vi "Measure4.vi"() -> ()   [LabVIEW 2024]
uses:
  <vilib>/MakerHub/LINX/Public/Peripherals/Analog/Analog Read N Chans.vi
  <vilib>/MakerHub/LINX/Public/Peripherals/PWM/PWM Set Duty Cycle 1 Chan.vi
  <vilib>/MakerHub/LINX/Public/Peripherals/Digital/Digital Read 1 Chan.vi
  <vilib>/MakerHub/LINX/Private/Local IO/LinxAnalogRead.vi
  <vilib>/MakerHub/LINX/Public/Utilities/Check Channel.vi
  <vilib>/MakerHub/LINX/Public/Peripherals/Digital/Digital Read N Chans.vi
  <vilib>/MakerHub/LINX/Private/Local IO/LinxDigitalRead.vi
  <vilib>/MakerHub/LINX/Public/Utilities/Open Serial.vi
  Globals.vi
  <vilib>/MakerHub/LINX/Public/Peripherals/PWM/PWM Set Duty Cycle N Chans.vi
  <vilib>/addons/control/pid/pid.llb/PID (DBL).vi
  <vilib>/MakerHub/LINX/Private/Utilties/Generate Error.vi
  <vilib>/Utility/file.llb/Write Delimited Spreadsheet (string).vi
  <vilib>/MakerHub/LINX/LMH-LINX.lvlib
  <vilib>/addons/control/pid/NI_PID_pid.lvlib
  <vilib>/Analysis/NI_AALBase.lvlib
panel:
  out "A5":dbl
  out "Resistance Amplified":dbl
  out "Resistance A3":dbl
  in  "Current":dbl
  out "A2 (TH)":dbl
  out "A1 (Voltage)":dbl
  out "A0 (TC)":dbl
  out "Resistance Amplified":dbl(graph)
  out "A4":dbl
  out "A3":dbl
  out "Resistance A3":dbl(graph)
  out "TREF 2 Error":dbl
  out "TREF 2":dbl
  out "TREF 1 Error":dbl
  out "Seebeck Coeff":dbl
  out "TREF 1":dbl
  in  "Target TC":dbl format="%.2f"
  in  "Target TH":dbl format="%.2f"
  out "Auto":bool
  in  "Start Auto":bool
  in  "TH End":dbl(knob)=100.0 step=10.0 scale=0.0..100.0
  in  "TH Start":dbl(knob)=40.0 step=10.0 scale=0.0..100.0
  out "VOUT - 1.25":dbl(knob) scale=-1.0..1.0
  out "TC":dbl(slide) scale=0.0..100.0
  out "TH":dbl(slide) scale=0.0..100.0
  out "Voltage":dbl(graph)
  out "TH":dbl(graph)
  in  "Save to File":bool
  out "VOUT - 1.25":dbl
  out "TC":dbl(graph)
  out "TC":dbl
  in  "Stop Button":bool
  out "TH":dbl
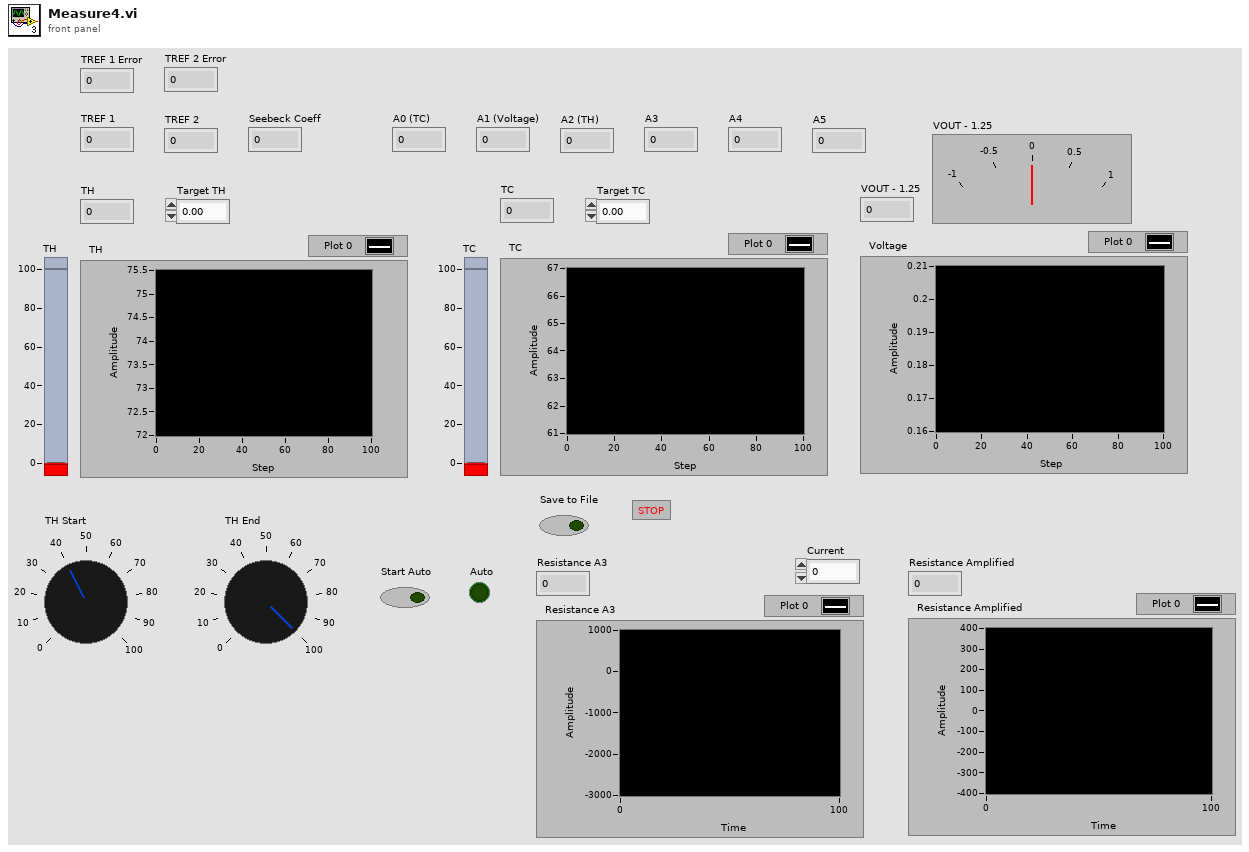
[diagram p1: front panel]
types:
  T1 = typedef "LMH-LINX.lvlib/LINX Ref.ctl" = cluster{"IO":T2, "Interface":T3, "LINX Device Config":T4}
  T2 = typedef "LMH-LINX.lvlib/Platform.ctl" = enum16{"Remote", "Local"}
  T3 = typedef "LMH-LINX.lvlib/Interface.ctl" = enum16{"Serial", "TCP"}
  T4 = typedef "LMH-LINX.lvlib/Device.lvlib/LINX Device Config.ctl" = cluster{"Interface":T3, "COM Port":refnum<visa-resource-name>, "TCP Configuration":T5, "Device Family":u8, "Device ID":u8, "Device Name":string, "TCP Ref":refnum<k5>, "Channels":T6}
  T5 = typedef "LMH-LINX.lvlib/Device.lvlib/TCP Config.ctl" = cluster{"IP Address":string, "Port":u16}
  T6 = typedef "LMH-LINX.lvlib/Channels.ctl" = cluster{"DI":u8[], "DO":u8[], "AI":u8[], "AO":u8[], "PWM":u8[], "QE":u8[], "UART":u8[], "I2C 2":u8[], "SPI":u8[], "CAN":u8[], "Servo":u8[], "AI Ref (V)":dbl, "AI Resolution (Bits)":u8, "AO Ref (V)":dbl, "AO Resolution (Bits)":u8}
  T7 = cluster{"proportional gain (Kc)":dbl, "integral time (Ti, min)":dbl, "derivative time (Td, min)":dbl}
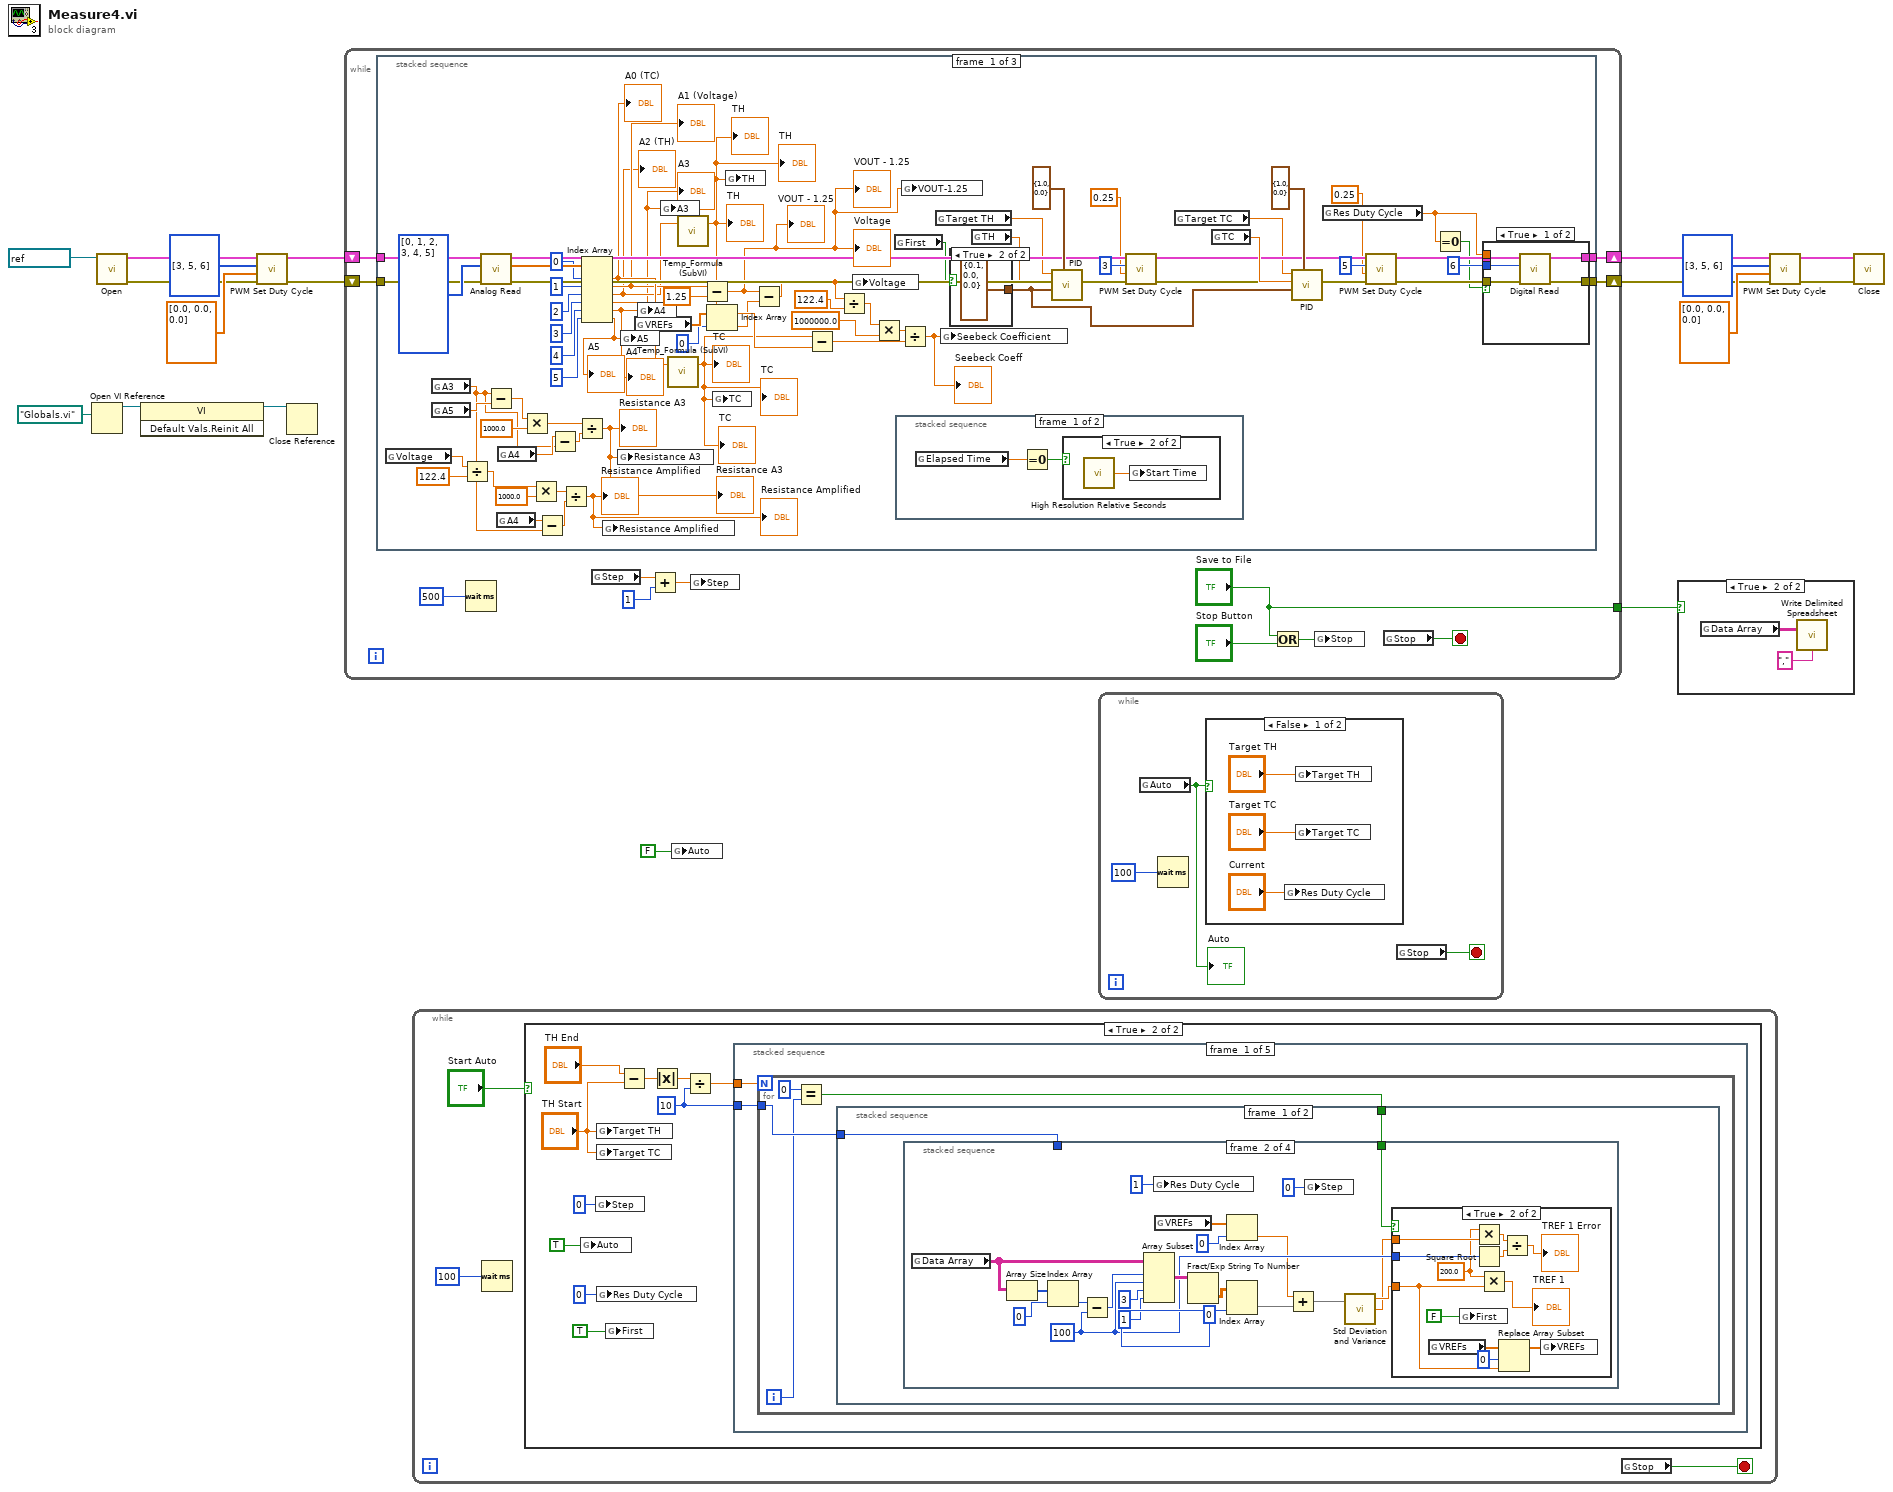
[diagram p0: block diagram]
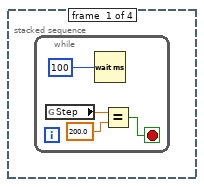
[diagram p3: hidden frame]
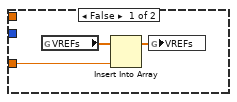
[diagram p4: hidden frame]
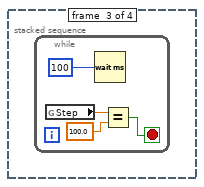
[diagram p5: hidden frame]
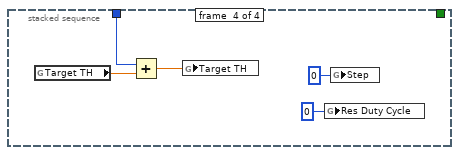
[diagram p6: hidden frame]
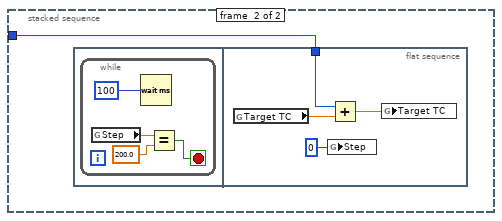
[diagram p7: hidden frame]
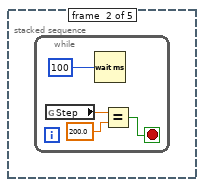
[diagram p8: hidden frame]
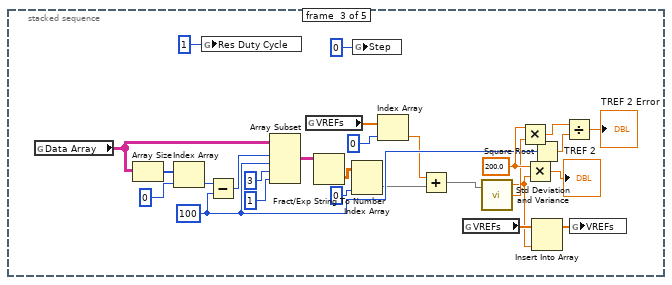
[diagram p9: hidden frame]
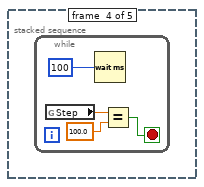
[diagram p10: hidden frame]
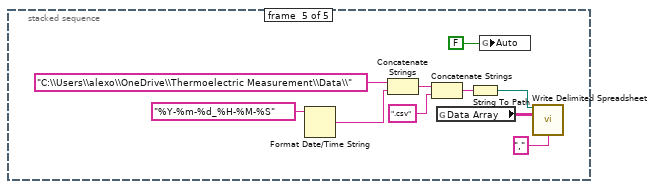
[diagram p11: hidden frame]
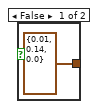
[diagram p14: hidden frame]
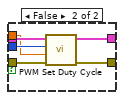
[diagram p15: hidden frame]
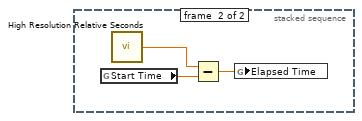
[diagram p17: hidden frame]
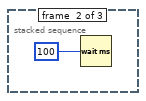
[diagram p18: hidden frame]
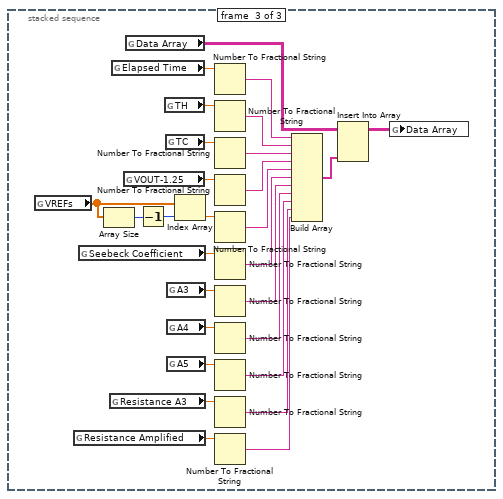
[diagram p19: hidden frame]
diagram:
  n1 = Open VI Reference(vi path=path "Globals.vi") -> (vi reference=w16:refnum<vi>)  [unwired: 5 in, 1 out]
  n2 = call-poly <vilib>:"Open.vi"("Serial Port"=refnum<visa-resource-name> "COM7") -> ("Error Out"=w8:errorcluster, "LINX Resource"=w11:T1)  [unwired: 8 in, 1 out]
  n3 = invoke class="VI" method="Default Vals.Reinit All"(reference=w16) -> (reference out=w15:refnum<vi>)  [unwired: 2 in, 2 out]
  n4 = call-poly <vilib>:"PWM Set Duty Cycle.vi"("Error In"=w8, "Duty Cycles"=dbl[] [0.0, 0.0, 0.0] ("Duty Cycle (0-1)"), "PWM Channels"=u8[] [3, 5, 6] ("PWM Channel"), "LINX Resource"=w11) -> ("Error Out"=w7:errorcluster, "LINX Resource"=w12:T1)  [unwired: 6 in]
  n5 = Close Reference(reference=w15) -> ()  [unwired: 1 in, 1 out]
  n6 = while {
    shift-right: [w29] -> w4
    shift-left: w12 -> [w30]
    shift-right: [w27] -> w1
    shift-left: w7 -> [w28]
    tunnel: ["Save to File"] -> w17
    stop <- w22 stop-if-true
    n7 = stacked-sequence {
      tunnel: w30 -> [w90 _ _]
      tunnel: [w56 _ _] -> w29
      tunnel: w28 -> [w89 _ _]
      tunnel: [w54 _ _] -> w27
      frame #0 {
        n8 = global read "Globals.vi" "Voltage"() -> (w52:dbl)
        n9 = global read "Globals.vi" "A3"() -> (w33:dbl)
        n10 = global read "Globals.vi" "A5"() -> (w41:dbl)
        n11 = Divide(x=w52, y=122.4) -> (x/y=w36:dbl)
        n12 = call-poly <vilib>:"Analog Read.vi"("Error In"=w89, "AI Channel(s)"=i32[] [0, 1, 2, 3, 4, 5], "LINX Resource"=w90) -> ("Error Out"=w87:errorcluster, "Voltages"=w96:dbl[], "LINX Resource"=w88:T1)  [unwired: 5 in, 1 out]
        n13 = Subtract(x=w33, y=w41) -> (x-y=w39:dbl)
        n14 = global read "Globals.vi" "A4"() -> (w37:dbl)
        n15 = global read "Globals.vi" "A4"() -> (w38:dbl)
        n16 = Multiply(x=w39, y=1000.0) -> (x*y=w67:dbl)
        n17 = Multiply(x=w36, y=1000.0) -> (x*y=w62:dbl)
        n18 = Subtract(x=w37, y=w33) -> (x-y=w61:dbl)
        n19 = Subtract(x=w38, y=w33) -> (x-y=w63:dbl)
        n20 = Divide(x=w62, y=w61) -> (x/y=w50:dbl)
        "Resistance Amplified" <- w50
        "Resistance Amplified" <- w50
        n21 = Divide(x=w67, y=w63) -> (x/y=w51:dbl)
        "Resistance A3" <- w51
        "Resistance A3" <- w51
        n22 = Index Array(array=w96, index #1=0 ("index"), index #2=1 ("index"), index #3=2 ("index"), index #4=3 ("index"), index #5=4 ("index"), index #6=5 ("index")) -> (element #1=w60:dbl, element #2=w59:dbl, element #3=w58:dbl, element #4=w48:dbl, element #5=w47:dbl, element #6=w43:dbl)
        "A3" <- w48
        "A4" <- w47
        "A0 (TC)" <- w60
        "A1 (Voltage)" <- w59
        "A2 (TH)" <- w58
        "A5" <- w43
        n23 = global write "Globals.vi" "Resistance Amplified"(w50) -> ()
        n24 = global write "Globals.vi" "Resistance A3"(w51) -> ()
        n25 = global write "Globals.vi" "A5"(w43) -> ()
        n26 = global read "Globals.vi" "VREFs"() -> (w71:dbl[])
        n27 = global write "Globals.vi" "A4"(w47) -> ()
        n28 = global write "Globals.vi" "A3"(w48) -> ()
        n29 = call "Temp_Formula (SubVI).vi"("In"=w60) -> ("Out"=w72:dbl)  [unwired: 1 in, 1 out]
        "TC" <- w72
        "TC" <- w72
        "TC" <- w72
        n30 = call "Temp_Formula (SubVI).vi"("In"=w58) -> ("Out"=w73:dbl)  [unwired: 1 in, 1 out]
        "TH" <- w73
        "TH" <- w73
        "TH" <- w73
        n31 = Subtract(x=w59, y=1.25) -> (x-y=w49:dbl)
        "VOUT - 1.25" <- w49
        "Voltage" <- w49
        "VOUT - 1.25" <- w49
        n32 = Index Array(array=w71, index=0) -> (element=w69:dbl)
        n33 = global write "Globals.vi" "TC"(w72) -> ()
        n34 = global write "Globals.vi" "TH"(w73) -> ()
        n35 = Subtract(x=w49, y=w69) -> (x-y=w68:dbl)
        n36 = Subtract(x=w72, y=w73) -> (x-y=w99:dbl)
        n37 = Divide(x=w68, y=122.4) -> (x/y=w74:dbl)
        n38 = global write "Globals.vi" "Voltage"(w68) -> ()
        n39 = Multiply(x=w74, y=1000000.0) -> (x*y=w77:dbl)
        n40 = global read "Globals.vi" "First"() -> (w35:bool)
        n41 = stacked-sequence {
          frame #0 {
            n42 = global read "Globals.vi" "Elapsed Time"() -> (w113:dbl)
            n43 = Equal To 0?(x=w113) -> (x = 0?=w114:bool)
            n44 = case shown="True" w114 {
              frame False {
              }
              frame True {
                n45 = call <vilib>:"High Resolution Relative Seconds.vi"() -> ("relative seconds"=w115:dbl)
                n46 = global write "Globals.vi" "Start Time"(w115) -> ()
              }
            }
          }
          frame #1 {
            n47 = global read "Globals.vi" "Start Time"() -> (w116:dbl)
            n48 = call <vilib>:"High Resolution Relative Seconds.vi"() -> ("relative seconds"=w117:dbl)
            n49 = Subtract(x=w117, y=w116) -> (x-y=w118:dbl)
            n50 = global write "Globals.vi" "Elapsed Time"(w118) -> ()
          }
        }
        n51 = Divide(x=w77, y=w99) -> (x/y=w98:dbl)
        "Seebeck Coeff" <- w98
        n52 = global write "Globals.vi" "VOUT-1.25"(w49) -> ()
        n53 = global read "Globals.vi" "Target TH"() -> (w80:dbl)
        n54 = global write "Globals.vi" "Seebeck Coefficient"(w98) -> ()
        n55 = case shown="True" w35 {
          tunnel: [T7 {"proportional gain (Kc)"=0.01, "integral time (Ti, min)"=0.14, "derivative time (Td, min)"=0.0} ("PID gains") T7 {"proportional gain (Kc)"=0.1, "integral time (Ti, min)"=0.0, "derivative time (Td, min)"=0.0} ("PID gains")] -> w34
          frame False {
          }
          frame True {
          }
        }
        n56 = global read "Globals.vi" "TH"() -> (w86:dbl)
        n57 = call-poly <vilib>:"PID.vi"("output range"=cluster{"output high":dbl, "output low":dbl} {"output high"=1.0, "output low"=0.0}, "PID gains"=w34, "process variable"=w86, "setpoint"=w80) -> ()  [unwired: 6 in, 2 out]
        n58 = call-poly <vilib>:"PWM Set Duty Cycle.vi"("Error In"=w87, "Duty Cycle (0-1)"=0.25, "PWM Channel"=u8 3, "LINX Resource"=w88) -> ("Error Out"=w81:errorcluster, "LINX Resource"=w82:T1)  [unwired: 6 in]
        n59 = global read "Globals.vi" "Target TC"() -> (w79:dbl)
        n60 = global read "Globals.vi" "TC"() -> (w83:dbl)
        n61 = call-poly <vilib>:"PID.vi"("output range"=cluster{"output high":dbl, "output low":dbl} {"output high"=1.0, "output low"=0.0}, "PID gains"=w34, "process variable"=w83, "setpoint"=w79) -> ()  [unwired: 6 in, 2 out]
        n62 = global read "Globals.vi" "Res Duty Cycle"() -> (w46:dbl)
        n63 = call-poly <vilib>:"PWM Set Duty Cycle.vi"("Error In"=w81, "Duty Cycle (0-1)"=0.25, "PWM Channel"=u8 5, "LINX Resource"=w82) -> ("Error Out"=w55:errorcluster, "LINX Resource"=w57:T1)  [unwired: 6 in]
        n64 = Equal To 0?(x=w46) -> (x = 0?=w45:bool)
        n65 = case shown="True" w45 {
          tunnel: w57 -> [w106 w112]
          tunnel: [w105 w111] -> w56
          tunnel: w55 -> [w103 w110]
          tunnel: [w104 w109] -> w54
          tunnel: u8 6 ("PWM Channel") -> [w102 w108]
          tunnel: w46 -> [_ w107]
          frame True {
            n66 = call-poly <vilib>:"Digital Read.vi"("Error In"=w103, "DI Channel"=w102, "LINX Resource"=w106) -> ("Error Out"=w104:errorcluster, "LINX Resource"=w105:T1)  [unwired: 6 in, 1 out]
          }
          frame False {
            n67 = call-poly <vilib>:"PWM Set Duty Cycle.vi"("Error In"=w110, "Duty Cycle (0-1)"=w107, "PWM Channel"=w108, "LINX Resource"=w112) -> ("Error Out"=w109:errorcluster, "LINX Resource"=w111:T1)  [unwired: 6 in]
          }
        }
      }
      frame #1 {
        n68 = Wait (ms)(milliseconds to wait=u32 100) -> ()  [unwired: 1 out]
      }
      frame #2 {
        n69 = global read "Globals.vi" "VREFs"() -> (w134:dbl[])
        n70 = global read "Globals.vi" "Resistance Amplified"() -> (w121:dbl)
        n71 = global read "Globals.vi" "Seebeck Coefficient"() -> (w138:dbl)
        n72 = Array Size(array=w134) -> (size(s)=w133:i32)
        n73 = global read "Globals.vi" "Resistance A3"() -> (w125:dbl)
        n74 = global read "Globals.vi" "Elapsed Time"() -> (w136:dbl)
        n75 = global read "Globals.vi" "VOUT-1.25"() -> (w143:dbl)
        n76 = global read "Globals.vi" "Data Array"() -> (w146:string[][])
        n77 = Decrement(x=w133) -> (x-1=w132:i32)
        n78 = global read "Globals.vi" "TH"() -> (w139:dbl)
        n79 = global read "Globals.vi" "TC"() -> (w141:dbl)
        n80 = global read "Globals.vi" "A3"() -> (w126:dbl)
        n81 = global read "Globals.vi" "A4"() -> (w127:dbl)
        n82 = global read "Globals.vi" "A5"() -> (w124:dbl)
        n83 = Index Array(array=w134, index=w132) -> (element=w131:dbl)
        n84 = Number To Fractional String(number=w136) -> (F-format string=w137:string)  [unwired: 3 in]
        n85 = Number To Fractional String(number=w139) -> (F-format string=w140:string)  [unwired: 3 in]
        n86 = Number To Fractional String(number=w141) -> (F-format string=w142:string)  [unwired: 3 in]
        n87 = Number To Fractional String(number=w143) -> (F-format string=w144:string)  [unwired: 3 in]
        n88 = Number To Fractional String(number=w131) -> (F-format string=w130:string)  [unwired: 3 in]
        n89 = Number To Fractional String(number=w138) -> (F-format string=w135:string)  [unwired: 3 in]
        n90 = Number To Fractional String(number=w126) -> (F-format string=w129:string)  [unwired: 3 in]
        n91 = Number To Fractional String(number=w127) -> (F-format string=w128:string)  [unwired: 3 in]
        n92 = Number To Fractional String(number=w124) -> (F-format string=w123:string)  [unwired: 3 in]
        n93 = Number To Fractional String(number=w125) -> (F-format string=w122:string)  [unwired: 3 in]
        n94 = Number To Fractional String(number=w121) -> (F-format string=w120:string)  [unwired: 3 in]
        n95 = Build Array(w137, w140, w142, w144, w130, w135, w129, w128, w123, w122, w120) -> (w145:string[])
        n96 = Insert Into Array(array=w146, new element=w145) -> (w147:string[][])  [unwired: 2 in]
        n97 = global write "Globals.vi" "Data Array"(w147) -> ()
      }
    }
    n98 = Wait (ms)(milliseconds to wait=u32 500) -> ()  [unwired: 1 out]
    n99 = global read "Globals.vi" "Step"() -> (w21:dbl)
    n100 = Add(x=w21, y=1) -> (x+y=w20:dbl)
    n101 = global write "Globals.vi" "Step"(w20) -> ()
    n102 = Or(x="Save to File", y="Stop Button") -> (x .or. y?=w23:bool)
    n103 = global write "Globals.vi" "Stop"(w23) -> ()
    n104 = global read "Globals.vi" "Stop"() -> (w22:bool)
  }
  n105 = while {
    stop <- w149 stop-if-true
    n106 = Wait (ms)(milliseconds to wait=u32 100) -> ()  [unwired: 1 out]
    n107 = case shown="True" "Start Auto" {
      frame False {
      }
      frame True {
        w155 = 10
        n108 = global write "Globals.vi" "Auto"(TRUE) -> ()
        n109 = global write "Globals.vi" "Step"(0) -> ()
        n110 = global write "Globals.vi" "Target TH"("TH Start") -> ()
        n111 = global write "Globals.vi" "Target TC"("TH Start") -> ()
        n112 = global write "Globals.vi" "Res Duty Cycle"(0) -> ()
        n113 = global write "Globals.vi" "First"(TRUE) -> ()
        n114 = Subtract(x="TH End", y="TH Start") -> (x-y=w158:dbl)
        n115 = Absolute Value(x=w158) -> (abs(x)=w157:dbl)
        n116 = Divide(x=w157, y=w155) -> (x/y=w154:dbl)
        n117 = stacked-sequence {
          tunnel: w154 -> [w162 _ _ _ _]
          tunnel: w155 -> [w161 _ _ _ _]
          frame #0 {
            n118 = for {
              N: w162 -> [_]
              tunnel: w161 -> [w166]
              i -> [w163]
              n119 = Equal?(x=0 ("y"), y=w163) -> (x = y?=w165:bool)
              n120 = stacked-sequence {
                tunnel: w166 -> [w168 w218]
                tunnel: w165 -> [w167 _]
                frame #0 {
                  n121 = stacked-sequence {
                    tunnel: w168 -> [_ _ _ w215]
                    tunnel: w167 -> [_ w193 _ _]
                    frame #0 {
                      n122 = while {
                        stop <- w169 stop-if-true
                        n123 = global read "Globals.vi" "Step"() -> (w171:dbl)
                        n124 = Wait (ms)(milliseconds to wait=u32 100) -> ()  [unwired: 1 out]
                        n125 = Equal?(x=w171, y=200.0) -> (x = y?=w169:bool)
                      }
                    }
                    frame #1 {
                      w181 = 100 ("y")
                      n126 = global read "Globals.vi" "Data Array"() -> (w187:string[][])
                      n127 = Array Size(array=w187) -> (size(s)=w188:i32[])
                      n128 = Index Array(array=w188, index=0) -> (element=w189:i32)
                      n129 = Subtract(x=w189, y=w181) -> (x-y=w190:i32)
                      n130 = Array Subset(array=w187, index (row)=w190, length (row)=w181, index (col)=3 ("index"), length (col)=1 ("length")) -> (w191:string[][])
                      n131 = global write "Globals.vi" "Res Duty Cycle"(1) -> ()
                      n132 = global read "Globals.vi" "VREFs"() -> (w179:dbl[])
                      n133 = Fract/Exp String To Number(string=w191) -> (number=w192:dbl[][])  [unwired: 3 in, 1 out]
                      n134 = Index Array(array=w179, index=0) -> (element=w177:dbl)
                      n135 = Index Array(array=w192, index (col)=0 ("dimension size")) -> (element=w175:dbl[])  [unwired: 1 in]
                      n136 = Add(x=w177, y=w175) -> (x+y=w176:dbl[])
                      n137 = global write "Globals.vi" "Step"(0) -> ()
                      n138 = call <vilib>:"Std Deviation and Variance.vi"("X"=w176) -> ("mean"=w182:dbl, "standard deviation"=w180:dbl)  [unwired: 1 in, 1 out]
                      n139 = case shown="True" w193 {
                        tunnel: w182 -> [w194 w199]
                        tunnel: w181 -> [_ w206]
                        tunnel: w180 -> [_ w205]
                        frame False {
                          n140 = global read "Globals.vi" "VREFs"() -> (w195:dbl[])
                          n141 = Insert Into Array(array=w195, new element=w194) -> (w196:dbl[])  [unwired: 1 in]
                          n142 = global write "Globals.vi" "VREFs"(w196) -> ()
                        }
                        frame True {
                          w202 = 200.0 ("x")
                          n143 = global read "Globals.vi" "VREFs"() -> (w201:dbl[])
                          n144 = global write "Globals.vi" "First"(FALSE) -> ()
                          n145 = Multiply(x=w202, y=w205) -> (x*y=w207:dbl)
                          n146 = Square Root(x=w206) -> (sqrt(x)=w203:dbl)
                          n147 = Multiply(x=w202, y=w199) -> (x*y=→"TREF 1":dbl)
                          n148 = Replace Array Subset(array=w201, new element=w199, index=0) -> (w200:dbl[])
                          n149 = Divide(x=w207, y=w203) -> (x/y=→"TREF 1 Error":dbl)
                          n150 = global write "Globals.vi" "VREFs"(w200) -> ()
                        }
                      }
                    }
                    frame #2 {
                      n151 = while {
                        stop <- w209 stop-if-true
                        n152 = global read "Globals.vi" "Step"() -> (w211:dbl)
                        n153 = Wait (ms)(milliseconds to wait=u32 100) -> ()  [unwired: 1 out]
                        n154 = Equal?(x=w211, y=100.0) -> (x = y?=w209:bool)
                      }
                    }
                    frame #3 {
                      n155 = global read "Globals.vi" "Target TH"() -> (w217:dbl)
                      n156 = Add(x=w215, y=w217) -> (x+y=w216:dbl)
                      n157 = global write "Globals.vi" "Target TH"(w216) -> ()
                      n158 = global write "Globals.vi" "Res Duty Cycle"(0) -> ()
                      n159 = global write "Globals.vi" "Step"(0) -> ()
                    }
                  }
                }
                frame #1 {
                  n160 = flat-sequence {
                    tunnel: w218 -> [w224]
                    frame #0 {
                      n161 = while {
                        stop <- w219 stop-if-true
                        n162 = global read "Globals.vi" "Step"() -> (w221:dbl)
                        n163 = Wait (ms)(milliseconds to wait=u32 100) -> ()  [unwired: 1 out]
                        n164 = Equal?(x=w221, y=200.0) -> (x = y?=w219:bool)
                      }
                    }
                    frame #1 {
                      n165 = global read "Globals.vi" "Target TC"() -> (w225:dbl)
                      n166 = global write "Globals.vi" "Step"(0) -> ()
                      n167 = Add(x=w224, y=w225) -> (x+y=w226:dbl)
                      n168 = global write "Globals.vi" "Target TC"(w226) -> ()
                    }
                  }
                }
              }
            }
          }
          frame #1 {
            n169 = while {
              stop <- w227 stop-if-true
              n170 = global read "Globals.vi" "Step"() -> (w229:dbl)
              n171 = Wait (ms)(milliseconds to wait=u32 100) -> ()  [unwired: 1 out]
              n172 = Equal?(x=w229, y=200.0) -> (x = y?=w227:bool)
            }
          }
          frame #2 {
            w248 = 200.0 ("x")
            w243 = 100 ("y")
            n173 = global read "Globals.vi" "Data Array"() -> (w257:string[][])
            n174 = Array Size(array=w257) -> (size(s)=w255:i32[])
            n175 = Index Array(array=w255, index=0) -> (element=w253:i32)
            n176 = global write "Globals.vi" "Res Duty Cycle"(1) -> ()
            n177 = Subtract(x=w253, y=w243) -> (x-y=w252:i32)
            n178 = Array Subset(array=w257, index (row)=w252, length (row)=w243, index (col)=3 ("index"), length (col)=1 ("length")) -> (w249:string[][])
            n179 = global read "Globals.vi" "VREFs"() -> (w237:dbl[])
            n180 = Fract/Exp String To Number(string=w249) -> (number=w242:dbl[][])  [unwired: 3 in, 1 out]
            n181 = Index Array(array=w242, index (col)=0 ("dimension size")) -> (element=w233:dbl[])  [unwired: 1 in]
            n182 = global write "Globals.vi" "Step"(0) -> ()
            n183 = Index Array(array=w237, index=0) -> (element=w235:dbl)
            n184 = Add(x=w235, y=w233) -> (x+y=w234:dbl[])
            n185 = global read "Globals.vi" "VREFs"() -> (w239:dbl[])
            n186 = call <vilib>:"Std Deviation and Variance.vi"("X"=w234) -> ("mean"=w238:dbl, "standard deviation"=w247:dbl)  [unwired: 1 in, 1 out]
            n187 = Multiply(x=w248, y=w247) -> (x*y=w246:dbl)
            n188 = Multiply(x=w248, y=w238) -> (x*y=→"TREF 2":dbl)
            n189 = Square Root(x=w243) -> (sqrt(x)=w245:dbl)
            n190 = Insert Into Array(array=w239, new element=w238) -> (w240:dbl[])  [unwired: 1 in]
            n191 = Divide(x=w246, y=w245) -> (x/y=→"TREF 2 Error":dbl)
            n192 = global write "Globals.vi" "VREFs"(w240) -> ()
          }
          frame #3 {
            n193 = while {
              stop <- w258 stop-if-true
              n194 = global read "Globals.vi" "Step"() -> (w260:dbl)
              n195 = Wait (ms)(milliseconds to wait=u32 100) -> ()  [unwired: 1 out]
              n196 = Equal?(x=w260, y=100.0) -> (x = y?=w258:bool)
            }
          }
          frame #4 {
            n197 = Format Date/Time String(time format string (%c)="%Y-%m-%d_%H-%M-%S") -> (date/time string=w266:string)  [unwired: 2 in]
            n198 = Concatenate Strings("C:\\Users\\alexo\\OneDrive\\Thermoelectric Measurement\\Data\\" ("string"), w266) -> (w267:string)
            n199 = Concatenate Strings(w267, ".csv" ("string")) -> (w264:string)
            n200 = global read "Globals.vi" "Data Array"() -> (w270:string[][])
            n201 = String To Path(string=w264) -> (path=w263:path)
            n202 = global write "Globals.vi" "Auto"(FALSE) -> ()
            n203 = call-poly <vilib>:"Write Delimited Spreadsheet.vi"("file path (dialog if empty)"=w263, "2D data"=w270, "delimiter (\\t)"="," ("delimiter (\\t)")) -> ()  [unwired: 11 in, 2 out]
          }
        }
      }
    }
    n204 = global read "Globals.vi" "Stop"() -> (w149:bool)
  }
  n205 = global write "Globals.vi" "Auto"(FALSE) -> ()
  n206 = while {
    stop <- w273 stop-if-true
    n207 = global read "Globals.vi" "Auto"() -> (w274:bool)
    "Auto" <- w274
    n208 = Wait (ms)(milliseconds to wait=u32 100) -> ()  [unwired: 1 out]
    n209 = case shown="False" w274 {
      frame False {
        n210 = global write "Globals.vi" "Res Duty Cycle"("Current") -> ()
        n211 = global write "Globals.vi" "Target TH"("Target TH") -> ()
        n212 = global write "Globals.vi" "Target TC"("Target TC") -> ()
      }
      frame True {
      }
    }
    n213 = global read "Globals.vi" "Stop"() -> (w273:bool)
  }
  n214 = case shown="True" w17 {
    frame False {
    }
    frame True {
      n215 = global read "Globals.vi" "Data Array"() -> (w279:string[][])
      n216 = call-poly <vilib>:"Write Delimited Spreadsheet.vi"("2D data"=w279, "delimiter (\\t)"="," ("delimiter (\\t)")) -> ()  [unwired: 12 in, 2 out]
    }
  }
  n217 = call-poly <vilib>:"PWM Set Duty Cycle.vi"("Error In"=w1, "Duty Cycles"=dbl[] [0.0, 0.0, 0.0] ("Duty Cycle (0-1)"), "PWM Channels"=u8[] [3, 5, 6] ("PWM Channel"), "LINX Resource"=w4) -> ("Error Out"=w2:errorcluster, "LINX Resource"=w3:T1)  [unwired: 6 in]
  n218 = call <vilib>:"Close.vi"("Error In"=w2, "LINX Resource"=w3) -> ()  [unwired: 9 in, 1 out]
